vi "to_json.vi"(8 "error in":errorcluster, 11 "ts.relative in":refnum<class "ts.relative.lvclass">) -> (0 "error out":errorcluster, 2 "json":string, 3 "ts.relative out":refnum<class "ts.relative.lvclass">, 4 "Not Default":bool)   [LabVIEW 2020, in "ts.relative.lvclass"]
uses:
  ts.relative.lvclass
  ts.relative.lvclass/ts.relative.ctl
  ac553a3d-6aa5-49ef-9e1c-caec14b63934.vi
  51cf98f5-1973-4989-a3e0-4cf140f0eb2f.vi
  <vilib>/LabVIEW Open Source Project/Epoch Date & Time/formatter.iso8601/Timestamp to ISO8601 UTC DateTime.vi
  <vilib>/JDP Science/JSONtext/Variant to JSON Text.vi
  <vilib>/JDP Science/JSONtext/LVClass Serializer/JSONtext LVClass Serializer.lvclass
  Nominal Client/Nominal Client.lvclass
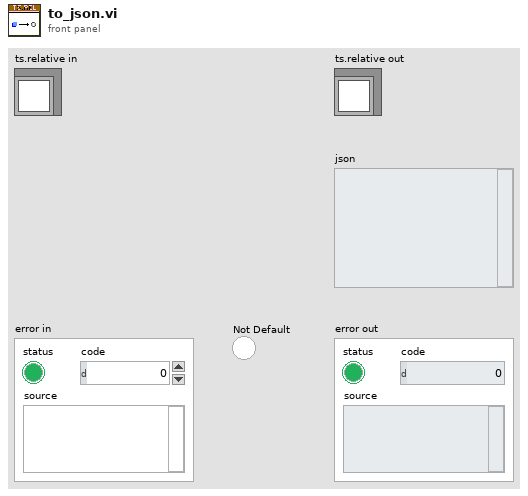
[diagram p1: front panel]
types:
  T1 = enum16{"DAYS", "HOURS", "MINUTES", "SECONDS", "MILLISECONDS", "MICROSECONDS", "NANOSECONDS", "PICOSECONDS"}
  T2 = cluster{"type":string, "relative":cluster{"timeUnit":string, "offset":string}}
  T3 = cluster{"type":string, "relative":cluster{"timeUnit":string}}
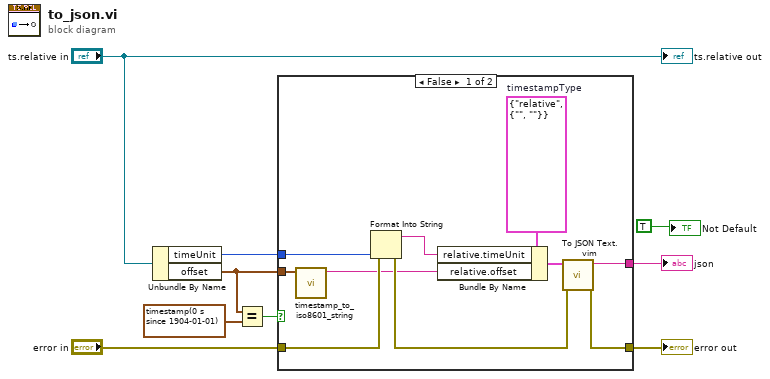
[diagram p0: block diagram]
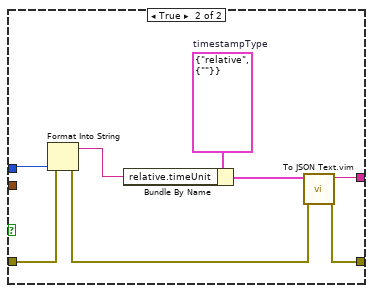
[diagram p2: hidden frame]
diagram:
  n1 = Unbundle By Name("ts.relative in") -> ("timeUnit"=w8:T1, "offset"=w7:timestamp)
  n2 = Equal?(x=w7, y=timestamp(0 s since 1904-01-01)) -> (x = y?=w5:bool)
  n3 = case shown="False" w5 {
    tunnel: w8 -> [w18 w24]
    tunnel: w7 -> [w19 _]
    tunnel: [w14 w23] -> w4
    tunnel: "error in" -> [w13 w22]
    tunnel: [w11 w20] -> w2
    frame False {
      w17 = T2 {"type"="relative", "relative"={"timeUnit"="", "offset"=""}}  # timestampType
      n4 = call "timestamp_to_iso8601_string.vi"("Time Stamp (now)"=w19) -> ("ISO8601 UTC DateTime"=w10:string)  [unwired: 10 in]
      n5 = Format Into String(error in=w13, w18) -> (resulting string=w16:string, error out=w12:errorcluster)  [unwired: 2 in]
      n6 = Bundle By Name(cluster=w17, "relative.timeUnit"=w16, "relative.offset"=w10) -> (w15:T2)
      n7 = call "To JSON Text.vim"("error in (no error)"=w12, "Anything"=w15) -> ("error out"=w11:errorcluster, "<JSON>"=w14:string)  [unwired: 8 in]
    }
    frame True {
      w27 = T3 {"type"="relative", "relative"={"timeUnit"=""}}  # timestampType
      n8 = Format Into String(error in=w22, w24) -> (resulting string=w26:string, error out=w21:errorcluster)  [unwired: 2 in]
      n9 = Bundle By Name(cluster=w27, "relative.timeUnit"=w26) -> (w25:T3)
      n10 = call "To JSON Text.vim"("error in (no error)"=w21, "Anything"=w25) -> ("error out"=w20:errorcluster, "<JSON>"=w23:string)  [unwired: 8 in]
    }
  }
  "error out" <- w2
  "json" <- w4
  "ts.relative out" <- "ts.relative in"
  "Not Default" <- TRUE
